vi "lvCICD.vi"(11 "CommandLine":string[](array[string])) -> (2 "test details":string, 3 "exit code":i32)   [LabVIEW 2014]
uses:
  <userlib>/_OpenG.lib/string/string.llb/Trim Whitespace (String Array)__ogtk.vi
  _lvcicd/_Strip apostrophe - array.vi
  <userlib>/_OpenG.lib/string/string.llb/Trim Whitespace (String)__ogtk.vi
  <userlib>/_OpenG.lib/string/string.llb/Convert EOLs (String)__ogtk.vi
  _lvcicd/_lvcicd_support.lvlib
panel:
  out "error out":errorcluster
  in  "error in (no error)":errorcluster
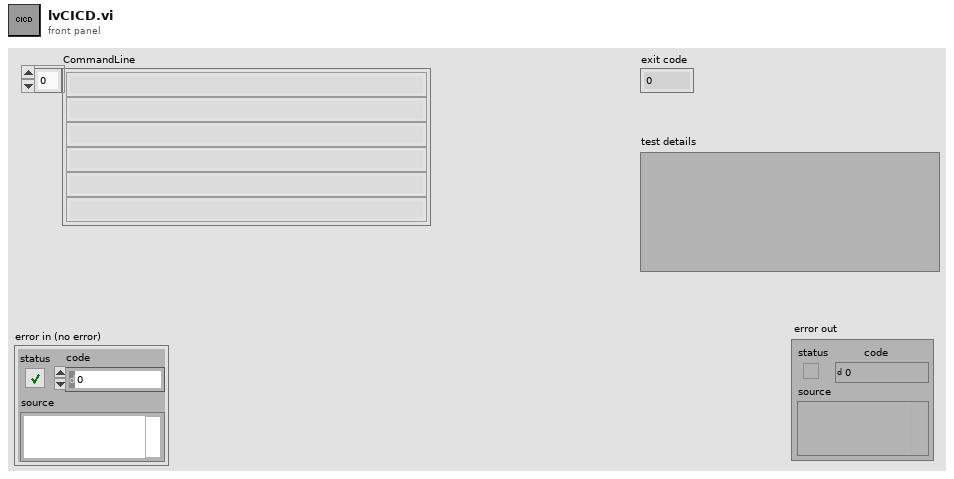
[diagram p1: front panel]
types:
  T1 = enum16{"open", "replace", "create", "open or create", "replace or create", "replace or create with confirmation"}
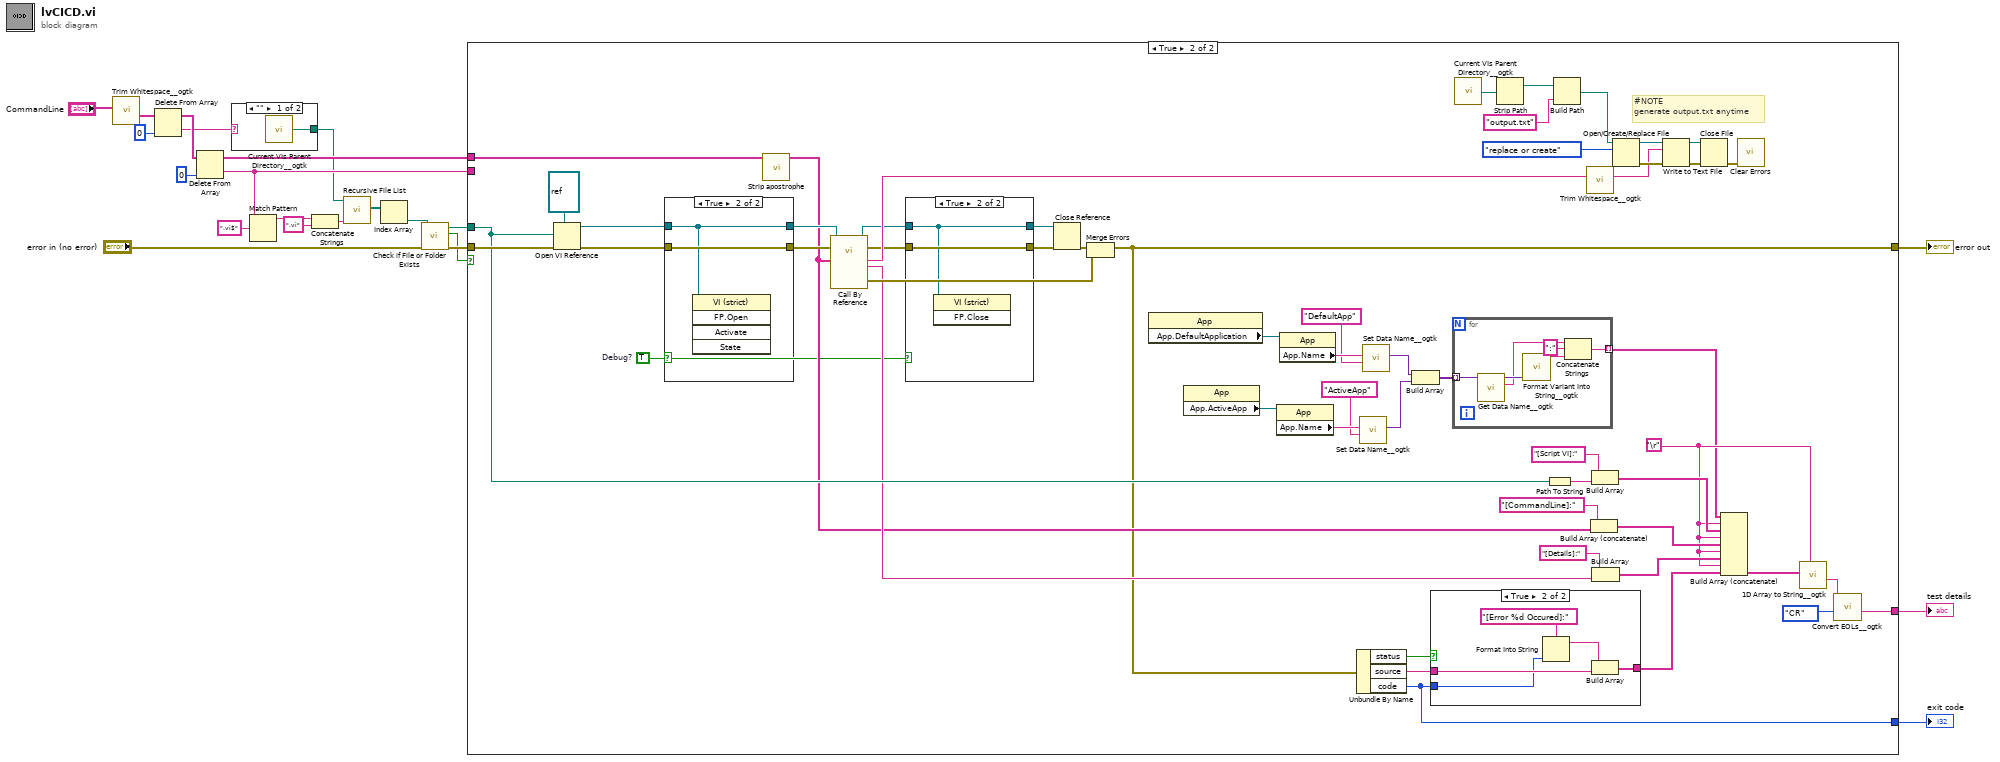
[diagram p0: block diagram]
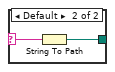
[diagram p2: hidden frame]
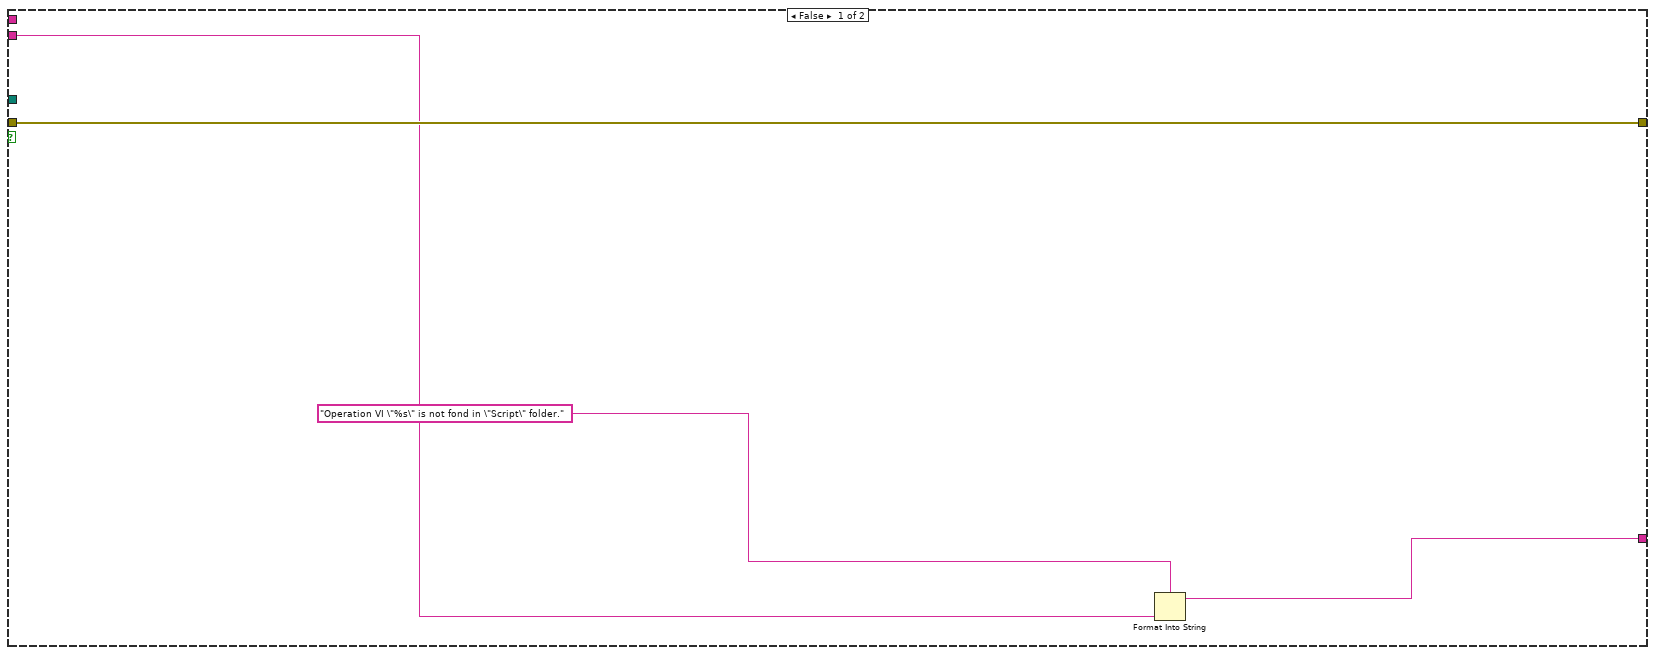
[diagram p3: hidden frame]
diagram:
  n1 = call-poly <userlib>:"Trim Whitespace__ogtk.vi"("String in"="CommandLine") -> ("String out"=w4:string[])  [unwired: 6 in]
  n2 = Delete From Array(array=w4, index=0) -> (deleted portion=w2:string, array with subset deleted=w3:string[])  [unwired: 1 in]
  n3 = Delete From Array(array=w3, index=0) -> (deleted portion=w6:string, array with subset deleted=w12:string[])  [unwired: 1 in]
  n4 = case shown="\"\"" w2 {
    selector: w2 -> [_ w25]
    tunnel: [w23 w24] -> w1
    frame "" {
      n5 = call <userlib>:"Current VIs Parent Directory__ogtk.vi"() -> ("Parent Directory (+ Relative)"=w23:path)  [unwired: 5 in]
    }
    frame Default {
      n6 = String To Path(string=w25) -> (path=w24:path)
    }
  }
  n7 = Match Pattern(string=w6, regular expression=".vi$") -> (before substring=w19:string)  [unwired: 1 in, 3 out]
  n8 = Concatenate Strings(w19, ".vi" ("string")) -> (w17:string)
  n9 = call <vilib>:"Recursive File List.vi"("pattern"=w17, "Folder Path"=w1) -> ("All Files in Dir"=w16:path[])  [unwired: 5 in, 4 out]
  n10 = Index Array(array=w16) -> (element=w15:path)  [unwired: 1 in]
  n11 = call <vilib>:"Check if File or Folder Exists.vi"("error in (no error)"="error in (no error)", "path"=w15) -> ("error out"=w14:errorcluster, "file or folder exists?"=w7:bool, "dup path"=w13:path)  [unwired: 7 in]
  n12 = case shown="True" w7 {
    tunnel: w14 -> [w29 w85]
    tunnel: w13 -> [_ w78]
    tunnel: w12 -> [_ w70]
    tunnel: [_ w48] -> w11
    tunnel: [w27 w80] -> w10
    tunnel: [w29 w46] -> w8
    tunnel: w6 -> [w26 _]
    frame False {
      n13 = Format Into String(format string="Operation VI \"%s\" is not fond in \"Script\" folder." ("String out"), w26) -> (resulting string=w27:string)  [unwired: 2 in, 1 out]
    }
    frame True {
      w30 = TRUE  # Debug?
      w44 = "\r"
      # "#NOTE\ngenerate output.txt anytime"
      n14 = Open VI Reference(type specifier VI Refnum (for type only)=refnum<vi> refnum, vi path=w78, error in (no error)=w85) -> (vi reference=w73:refnum<vi>, error out=w83:errorcluster)  [unwired: 3 in]
      n15 = case shown="True" w30 {
        tunnel: w83 -> [w101 w104]
        tunnel: [w101 w104] -> w74
        tunnel: w73 -> [w102 w103]
        tunnel: [w102 w103] -> w72
        frame False {
        }
        frame True {
          n16 = invoke class="VI (strict)" method="FP.Open"(reference=w103) -> ()  [unwired: 4 in, 5 out]
        }
      }
      n17 = call-poly "Strip apostrophe.vi"("string"=w70) -> ("content"=w61:string[])  [unwired: 10 in]
      n18 = call-by-ref "?"(reference=w72, error in=w74, "CommandLine"=w61) -> (reference out=w32:refnum<vi>, error out=w34:errorcluster, 0:"error out"=w81:errorcluster, "test details"=w64:string, "output to action"=w60:string)  [unwired: 8 in]
      n19 = case shown="True" w30 {
        tunnel: w34 -> [w86 w89]
        tunnel: [w86 w89] -> w33
        tunnel: w32 -> [w87 w88]
        tunnel: [w87 w88] -> w31
        frame False {
        }
        frame True {
          n20 = invoke class="VI (strict)" method="FP.Close"(reference=w88) -> ()  [unwired: 2 in, 3 out]
        }
      }
      n21 = Close Reference(reference=w31, error in (no error)=w33) -> (error out=w82:errorcluster)
      n22 = Merge Errors(w82, w81) -> (w46:errorcluster)
      n23 = property class="App"() -> ("App.DefaultApplication"=w40:refnum<vi>)  [unwired: 2 in, 2 out]
      n24 = property class="App"() -> ("App.ActiveApp"=w39:refnum<vi>)  [unwired: 2 in, 2 out]
      n25 = property class="App"(reference=w39) -> ("App.Name"=w41:string)  [unwired: 1 in, 2 out]
      n26 = property class="App"(reference=w40) -> ("App.Name"=w42:string)  [unwired: 1 in, 2 out]
      n27 = Unbundle By Name(w46) -> ("status"=w49:bool, "source"=w77:string, "code"=w48:i32)
      n28 = call <userlib>:"Set Data Name__ogtk.vi"("Data Name"="ActiveApp", "Data"=w41) -> ("Renamed Data"=w35:variant)  [unwired: 8 in, 1 out]
      n29 = call <userlib>:"Set Data Name__ogtk.vi"("Data Name"="DefaultApp", "Data"=w42) -> ("Renamed Data"=w36:variant)  [unwired: 8 in, 1 out]
      n30 = Build Array(w36, w35) -> (w45:variant[])
      n31 = case shown="True" w49 {
        tunnel: w77 -> [_ w100]
        tunnel: [_ w99] -> w76
        tunnel: w48 -> [_ w98]
        frame False {
        }
        frame True {
          n32 = Format Into String(format string="[Error %d Occured]:" ("element"), w98) -> (resulting string=w96:string)  [unwired: 2 in, 1 out]
          n33 = Build Array(w96, w100) -> (w99:string[])
        }
      }
      n34 = for {
        tunnel: w45 -> [w95] mode=indexing
        tunnel: [w90] -> w43 mode=indexing
        n35 = call <userlib>:"Get Data Name__ogtk.vi"("Data"=w95) -> ("Data Name"=w92:string, "Data dup"=w94:variant)  [unwired: 8 in, 1 out]
        n36 = call <userlib>:"Format Variant Into String__ogtk.vi"("Variant"=w94) -> ("Output String"=w93:string)  [unwired: 13 in, 1 out]
        n37 = Concatenate Strings(w92, ":" ("string"), w93) -> (w90:string)
      }
      n38 = call <userlib>:"Current VIs Parent Directory__ogtk.vi"() -> ("Parent Directory (+ Relative)"=w58:path)  [unwired: 5 in]
      n39 = Strip Path(path=w58) -> (stripped path=w59:path)  [unwired: 1 out]
      n40 = Path To String(path=w78) -> (string=w68:string)
      n41 = Build Path(base path=w59, name or relative path="output.txt") -> (appended path=w56:path)
      n42 = call-poly <userlib>:"Trim Whitespace__ogtk.vi"("String in"=w60) -> ("String out"=w50:string)  [unwired: 6 in]
      n43 = Build Array (concatenate)("[CommandLine]:" ("element"), w61) -> (w66:string[])
      n44 = Build Array("[Script VI]:" ("element"), w68) -> (w67:string[])
      n45 = Build Array("[Details]:" ("element"), w64) -> (w63:string[])
      n46 = Open/Create/Replace File(file path (use dialog)=w56, operation (0:open)=T1."replace or create") -> (refnum out=w54:refnum<file>, error out=w55:errorcluster)  [unwired: 4 in, 1 out]
      n47 = Write to Text File(file (use dialog)=w54, text=w50, error in=w55) -> (refnum out=w52:refnum<file>, error out=w53:errorcluster)  [unwired: 1 in, 1 out]
      n48 = Close File(refnum=w52, error in=w53) -> (error out=w47:errorcluster)  [unwired: 1 out]
      n49 = Build Array (concatenate)(w43, w44, w67, w44, w66, w44, w63, w44, w76) -> (w62:string[])
      n50 = call <vilib>:"Clear Errors.vi"("error in (no error)"=w47) -> ()  [unwired: 5 in, 2 out]
      n51 = call <userlib>:"1D Array to String__ogtk.vi"("delimiter (Tab)"=w44, "Array of Strings"=w62) -> ("delimited string"=w75:string)  [unwired: 9 in]
      n52 = call-poly <userlib>:"Convert EOLs__ogtk.vi"("Convert to:"=enum16{"CR", "LF", "CRLF"}."CR", "String in"=w75) -> ("String out"=w80:string)  [unwired: 9 in]
    }
  }
  "test details" <- w10
  "exit code" <- w11
  "error out" <- w8
